vi "Run VI Tester.vi"(0 "test path":path, 11 "error in":errorcluster) -> (4 "successful?":bool, 6 "test details":string, 15 "error out":errorcluster)   [LabVIEW 2026]
doc: "Runs every test of a VI Tester test case class or suite through JKI's own programmatic API (Run Tests (Path).vi) - no dialog - and returns whether all passed and the text report."
uses:
  <vilib>/addons/_JKI Toolkits/VI Tester/VI Tester API.llb/VI Tester API.lvlib
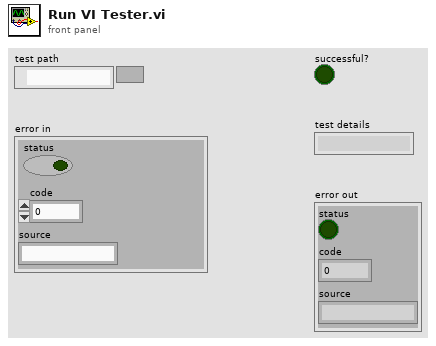
[diagram p1: front panel]
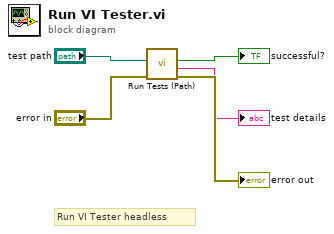
[diagram p0: block diagram]
diagram:
  # "Run VI Tester headless"
  n1 = call <vilib>:"Run Tests (Path).vi"("error in (no error)"="error in", "Test Path"="test path") -> ("error out"=→"error out":errorcluster, "test details"=→"test details":string, "successful?"=→"successful?":bool)  [unwired: 7 in]
